vi "RemoteVI Status Text.vi"(0 "status":T1(array[cluster])) -> (4 "text":string)   [LabVIEW 2020, in "RemoteVI.lvlib"]
doc: "Writes the status RemoteVI Status.vi returns as text, one block per share, lines joined with a line feed: Port 8088: RemoteVI Demo.vi (VI), running for 1 min 5 s, this computer only (, view only); the link; clients, fps, kB/s, frames and the input-to-frame latency; one line per client (address, connected for, last input); the last error if there is one. No share: No RemoteVI share is running. Numbers are written with a decimal point whatever the system's locale. Pure function, cannot fail. Reference: statusText() in tools\\lib\\status.mjs, vectors tests\\vectors\\status.json (texts)."
uses:
  RemoteVI.lvlib
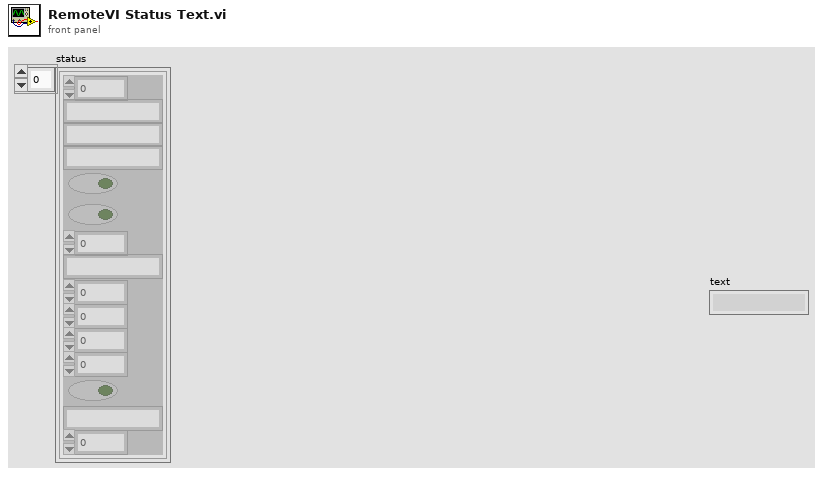
[diagram p1: front panel]
types:
  T1 = cluster{"port":u16, "url":string, "target":string, "kind":string, "whole network":bool, "running":bool, "uptime s":dbl, "clients":cluster{"address":string, "connected s":dbl, "idle s":dbl}[], "fps":dbl, "kB per s":dbl, "frames":u32, "latency ms":dbl, "view only":bool, "last error":string, "hWnd":u64}[]
  T2 = cluster{"address":string, "connected s":dbl, "idle s":dbl}[]
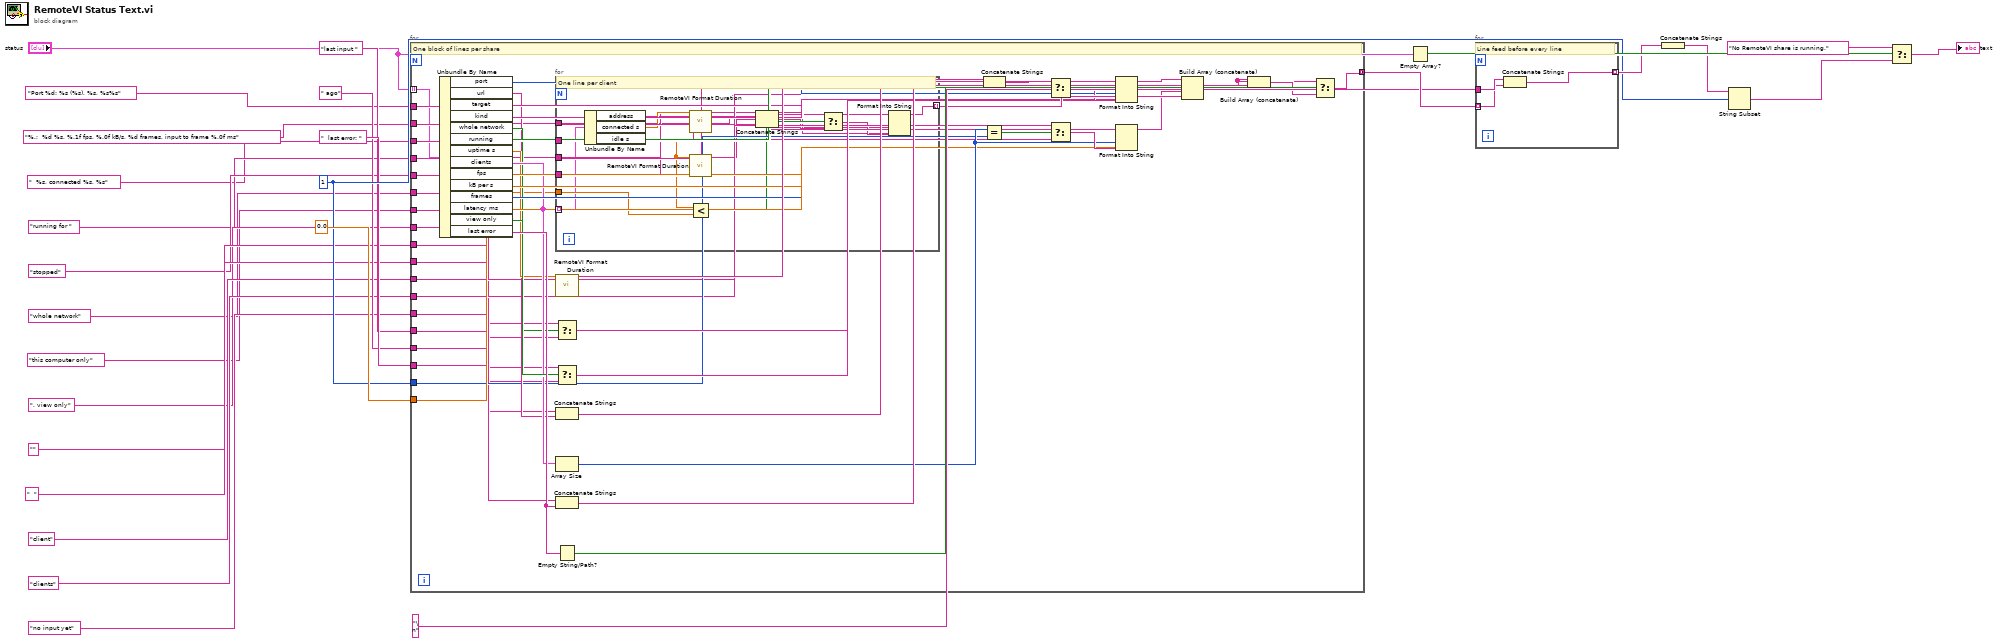
[diagram p0: block diagram]
diagram:
  w20 = 1
  n1 = for {
    tunnel: "status" -> [w28] mode=indexing
    tunnel: "Port %d: %s (%s), %s, %s%s" -> [w29]
    tunnel: "%.;  %d %s, %.1f fps, %.0f kB/s, %d frames, input to frame %.0f ms" -> [w30]
    tunnel: "  %s, connected %s, %s" -> [w31]
    tunnel: "running for " -> [w32]
    tunnel: "stopped" -> [w33]
    tunnel: "whole network" -> [w34]
    tunnel: "this computer only" -> [w35]
    tunnel: ", view only" -> [w36]
    tunnel: "" -> [w37]
    tunnel: "  " -> [w38]
    tunnel: "client" -> [w39]
    tunnel: "clients" -> [w40]
    tunnel: "no input yet" -> [w41]
    tunnel: "last input " -> [w42]
    tunnel: " ago" -> [w43]
    tunnel: "  last error: " -> [w44]
    tunnel: w20 -> [w45]
    tunnel: 0.0 -> [w46]
    tunnel: [w77] -> w22 mode=concatenating
    # "One block of lines per share"
    n2 = Unbundle By Name(w28) -> ("port"=w47:u16, "url"=w48:string, "target"=w49:string, "kind"=w50:string, "whole network"=w51:bool, "running"=w52:bool, "uptime s"=w53:dbl, "clients"=w54:T2, "fps"=w55:dbl, "kB per s"=w56:dbl, "frames"=w57:u32, "latency ms"=w58:dbl, "view only"=w59:bool, "last error"=w60:string)
    n3 = for {
      tunnel: w31 -> [w79]
      tunnel: w41 -> [w80]
      tunnel: w42 -> [w81]
      tunnel: w43 -> [w82]
      tunnel: w46 -> [w83]
      tunnel: w54 -> [w78] mode=indexing
      tunnel: [w92] -> w72 mode=indexing
      # "One line per client"
      n4 = Unbundle By Name(w78) -> ("address"=w84:string, "connected s"=w85:dbl, "idle s"=w86:dbl)
      n5 = call "RemoteVI Format Duration.vi"("seconds"=w85) -> ("text"=w87:string)  [unwired: 14 in]
      n6 = call "RemoteVI Format Duration.vi"("seconds"=w86) -> ("text"=w88:string)  [unwired: 14 in]
      n7 = Less?(x=w86, y=w83) -> (x < y?=w90:bool)
      n8 = Concatenate Strings(w81, w88, w82) -> (w89:string)
      n9 = Select(t=w80, s=w90, f=w89) -> (s? t:f=w91:string)
      n10 = Format Into String(format string=w79, w84, w87, w91) -> (resulting string=w92:string)  [unwired: 2 in, 1 out]
    }
    n11 = call "RemoteVI Format Duration.vi"("seconds"=w53) -> ("text"=w61:string)  [unwired: 14 in]
    n12 = Select(t=w34, s=w51, f=w35) -> (s? t:f=w64:string)
    n13 = Select(t=w36, s=w59, f=w37) -> (s? t:f=w65:string)
    n14 = Concatenate Strings(w38, w48) -> (w67:string)
    n15 = Array Size(array=w54) -> (size(s)=w68:i32)
    n16 = Concatenate Strings(w44, w60) -> (w74:string)
    n17 = Empty String/Path?(string/path=w60) -> (empty?=w76:bool)
    n18 = Concatenate Strings(w32, w61) -> (w62:string)
    n19 = Equal?(x=w68, y=w45) -> (x = y?=w69:bool)
    n20 = Select(t=w62, s=w52, f=w33) -> (s? t:f=w63:string)
    n21 = Select(t=w39, s=w69, f=w40) -> (s? t:f=w70:string)
    n22 = Format Into String(format string=w29, w47, w49, w50, w63, w64, w65) -> (resulting string=w66:string)  [unwired: 2 in, 1 out]
    n23 = Format Into String(format string=w30, w68, w70, w55, w56, w57, w58) -> (resulting string=w71:string)  [unwired: 2 in, 1 out]
    n24 = Build Array (concatenate)(w66, w67, w71, w72) -> (w73:string[])
    n25 = Build Array (concatenate)(w73, w74) -> (w75:string[])
    n26 = Select(t=w73, s=w76, f=w75) -> (s? t:f=w77:string[])
  }
  n27 = Empty Array?(array="status") -> (empty?=w26:bool)
  n28 = for {
    tunnel: "\n" -> [w94]
    tunnel: w22 -> [w93] mode=indexing
    tunnel: [w95] -> w23 mode=indexing
    # "Line feed before every line"
    n29 = Concatenate Strings(w94, w93) -> (w95:string)
  }
  n30 = Concatenate Strings(w23) -> (w24:string)
  n31 = String Subset(string=w24, offset (0)=w20) -> (substring=w25:string)  [unwired: 1 in]
  n32 = Select(t="No RemoteVI share is running.", s=w26, f=w25) -> (s? t:f=→"text":string)
